vi "Test Performance.vi"() -> ()   [LabVIEW 2019]
uses:
  src/xy_utilities.lvlib
  <vilib>/Analysis/NI_AALBase.lvlib
  <vilib>/Analysis/baseanly.llb/Mean (DBL).vi
panel:
  out "XY Data 3":cluster{"X-array":dbl[], "Y-array":dbl[]}[](graph)
  out "Intensity Graph 2":dbl[][](graph)
  out "Intensity Graph":dbl[][](graph)
  out "execution time (s)":dbl
  out "XY Data 2":cluster{"X-array":dbl[], "Y-array":dbl[]}(graph)
  out "XY Data":cluster{"X-array":dbl[], "Y-array":dbl[]}[](graph)
  # "0: 21\"\n5: 0.09\""
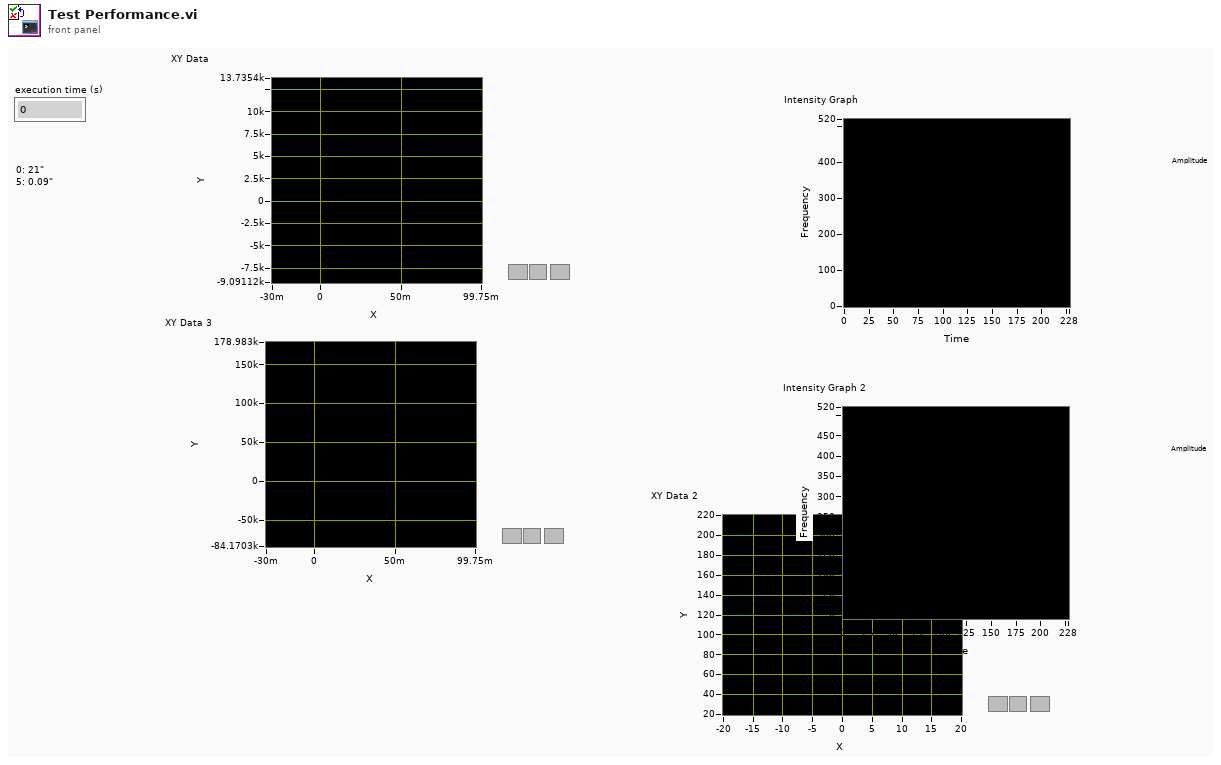
[diagram p1: front panel]
types:
  T1 = enum16{"thermal waveguide", "superlattice waveguide", "decay in atmosphere"}
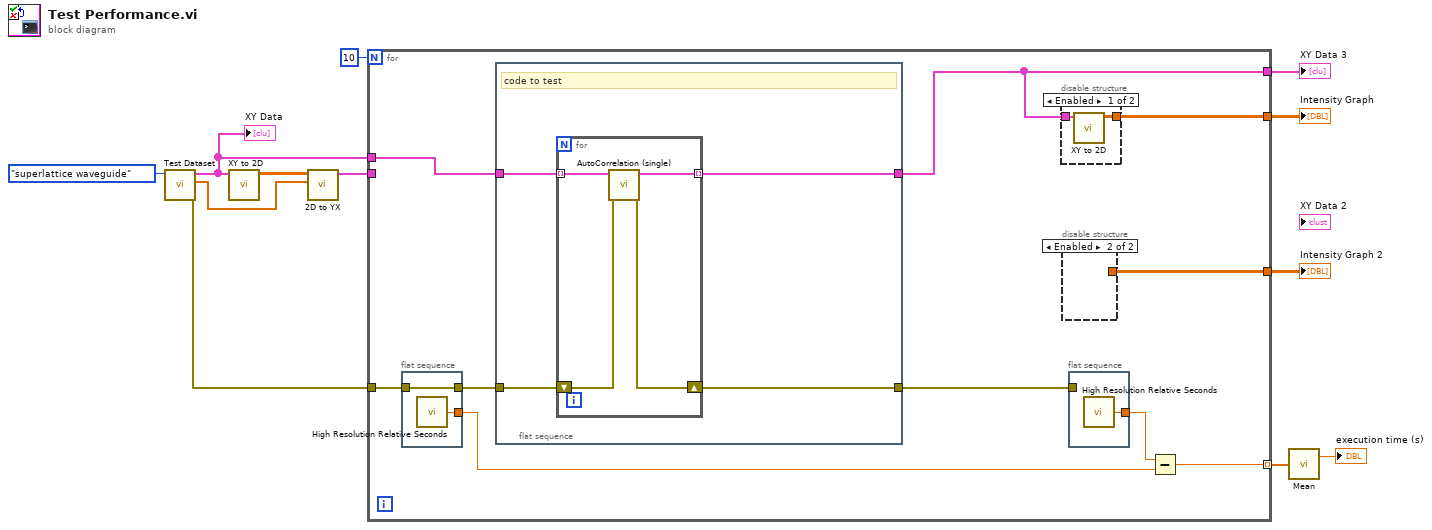
[diagram p0: block diagram]
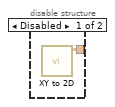
[diagram p2: hidden frame]
diagram:
  n1 = call "Test Dataset.vi"("Enum"=T1."superlattice waveguide") -> ("error out"=w12:errorcluster, "Parameters out"=w7:dbl[], "XY-data out"=w2:cluster{"X-array":dbl[], "Y-array":dbl[]}[])  [unwired: 8 in]
  "XY Data" <- w2
  n2 = call "XY to 2D.vi"("XY-data"=w2) -> ("2D Z Array"=w6:dbl[][])  [unwired: 7 in, 3 out]
  n3 = call "2D to YX.vi"("Y Array"=w7, "2D Z Array"=w6) -> ("XY-data out"=w5:cluster{"X-array":dbl[], "Y-array":dbl[]}[])  [unwired: 8 in, 1 out]
  n4 = for {
    N: 10 -> [_]
    tunnel: w12 -> [w22]
    tunnel: w5 -> [_]
    tunnel: [w19] -> w11
    tunnel: [w18] -> w10
    tunnel: [w15] -> w8 mode=indexing
    tunnel: [w14] -> w4
    tunnel: w2 -> [w13]
    n5 = flat-sequence {
      tunnel: [w36] -> w17
      tunnel: w22 -> [w36]
      tunnel: [w35] -> w20
      frame #0 {
        n6 = call <vilib>:"High Resolution Relative Seconds.vi"() -> ("relative seconds"=w35:dbl)
      }
    }
    n7 = flat-sequence {
      tunnel: w13 -> [w29]
      tunnel: w17 -> [w27]
      tunnel: [w26] -> w16
      tunnel: [w28] -> w14
      frame #0 {
        # "code to test"
        n8 = for {
          tunnel: w29 -> [w33] mode=indexing
          tunnel: [w32] -> w28 mode=indexing
          shift-right: [w30] -> w26
          shift-left: w27 -> [w31]
          n9 = call "AutoCorrelation (single).vi"("error in (no error)"=w31, "XY-data a"=w33) -> ("error out"=w30:errorcluster, "XY-data a out"=w32:cluster{"X-array":dbl[], "Y-array":dbl[]})  [unwired: 8 in]
        }
      }
    }
    n10 = disable-structure shown="Enabled" {
      disable-tunnel: [w25 _] -> w18
      disable-tunnel: w14 -> [w24 _]
      frame Enabled {
        n11 = call "XY to 2D.vi"("XY-data"=w24) -> ("2D Z Array"=w25:dbl[][])  [unwired: 7 in, 3 out]
      }
      frame Disabled {
      }
    }
    n12 = disable-structure shown="Enabled" {
      disable-tunnel: [w23 _] -> w19
      frame Disabled {
        n13 = call "XY to 2D.vi"() -> ("2D Z Array"=w23:dbl[][])  [unwired: 8 in, 3 out]
      }
      frame Enabled {
      }
    }
    n14 = flat-sequence {
      tunnel: [w34] -> w21
      tunnel: w16 -> [_]
      frame #0 {
        n15 = call <vilib>:"High Resolution Relative Seconds.vi"() -> ("relative seconds"=w34:dbl)
      }
    }
    n16 = Subtract(x=w21, y=w20) -> (x-y=w15:dbl)
  }
  "Intensity Graph" <- w10
  "Intensity Graph 2" <- w11
  "XY Data 3" <- w4
  n17 = call-poly <vilib>:"Mean.vi"("X"=w8) -> ("mean"=→"execution time (s)":dbl)  [unwired: 1 out]
